vi "bnal PLOT_NS.vi"(7 "AS IDX":i32[](array[numeric]), 8 "error in":errorcluster caption="エラー入力（エラーなし）", 9 "Signal Intensity [pA]":dbl[](array[numeric]), 10 "Time":dbl[](array[numeric]), 11 "Relative Averaged Data":dbl[](array[numeric])) -> (0 "error out":errorcluster caption="エラー出力", 1 "R Con H":dbl[][](array[numeric]), 2 "Plot_C":T2, 3 "Plot Graph":T1)   [LabVIEW 2018]
uses:
  <vilib>/Analysis/NI_AALPro.lvlib
  <vilib>/Analysis/NI_AALBase.lvlib
panel:
  out "x/y":dbl
  out "New MIN":dbl
  out "New MAX 2":dbl
  out "最大値 2":dbl
  out "Histogram":i32[][](array[numeric])
  out "配列 2":dbl[][](array[numeric])
  out "GAT":T3
  out "GAF":T4
  out "Abs MIN 2":dbl
  out "Abs MAX 2":dbl
  out "Axis 2":dbl[](array[numeric])
  out "Abs MIN":dbl
  out "Abs MAX":dbl
  out "Axis":dbl[](array[numeric]) caption="軸" format="%0.2f"
  out "Abs Plot Graph":dbl[][](graph)
  out "Abs Average":dbl[](array[numeric])
  out "Total Con and T":T5
  out "T STD (%)":dbl[](array[numeric])
  out "T Average":dbl[](array[numeric])
  out "New bin":dbl
  out "New MAX":dbl
  out "Count Graph":cluster{i32[], i32[]}(graph) caption="ヒストグラムグラフ"
  out "Normalized Plot Graph":dbl[][](graph)
  out "STD (%)":dbl[](array[numeric])
  out "Average":dbl[](array[numeric])
  out "layer":i32[](array[numeric])
  out "Plot Graph":dbl[][](graph)
  out "配列":dbl[](array[numeric])
  out "Histogram 2":i32[](array[numeric]) caption="ヒストグラム"
  out "最大値":i32
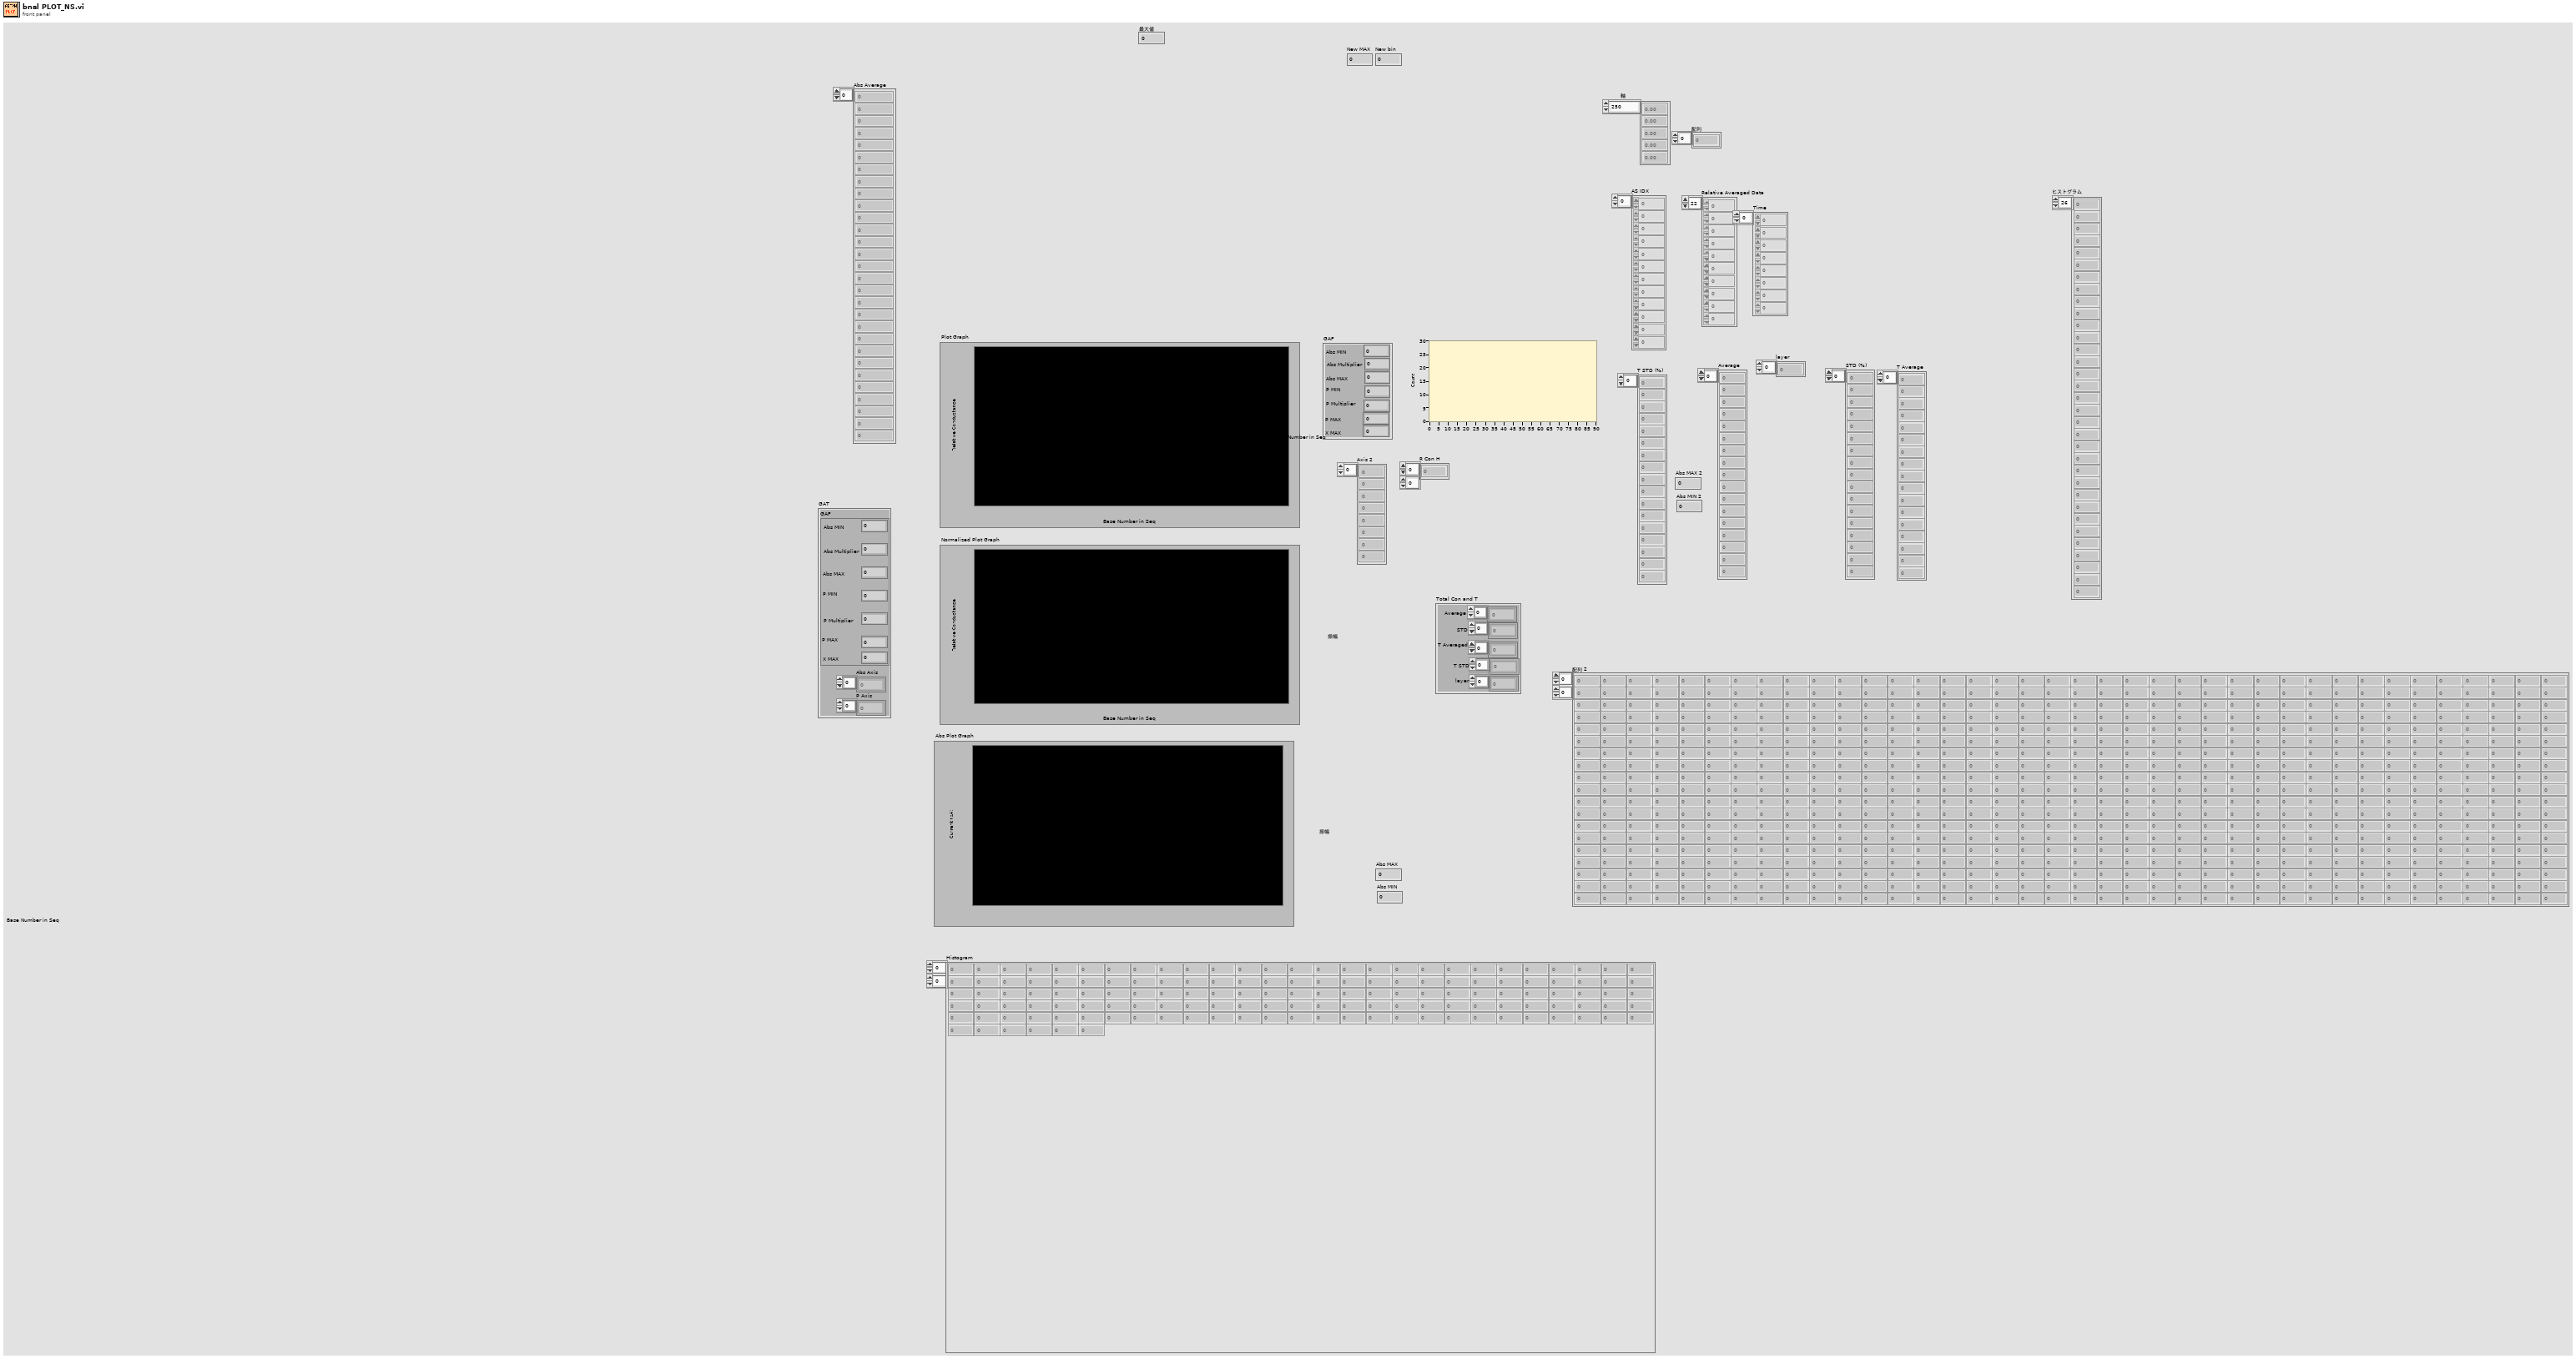
[diagram p1: front panel]
types:
  T1 = cluster{"Plot Graph":dbl[][], "N_Grpah":dbl[][], "Abs_Graph":dbl[][]}
  T2 = cluster{"Count Graph":cluster{i32[], i32[]}, "Total Con and T":cluster{dbl[], dbl[], dbl[], dbl[], i32[]}, "GAT":cluster{"Value":cluster{"Abs MIN":dbl, "Abs Multiplier":dbl, "Abs MAX":dbl, "P MIN":dbl, "P Multiplier":dbl, "P MAX":dbl, "X MAX":dbl}, "Axis":dbl[], "Axis":dbl[]}}
  T3 = cluster{"GAF":cluster{"Abs MIN":dbl, "Abs Multiplier":dbl, "Abs MAX":dbl, "P MIN":dbl, "P Multiplier":dbl, "P MAX":dbl, "X MAX":dbl}, "Abs Axis":dbl[], "P Axis":dbl[]}
  T4 = cluster{"Abs MIN":dbl, "Abs Multiplier":dbl, "Abs MAX":dbl, "P MIN":dbl, "P Multiplier":dbl, "P MAX":dbl, "X MAX":dbl}
  T5 = cluster{"Average":dbl[], "STD":dbl[], "T Averaged":dbl[], "T STD":dbl[], "layer":i32[]}
  T6 = cluster{"Value":cluster{"Abs MIN":dbl, "Abs Multiplier":dbl, "Abs MAX":dbl, "P MIN":dbl, "P Multiplier":dbl, "P MAX":dbl, "X MAX":dbl}, "Axis":dbl[], "Axis":dbl[]}
  T7 = cluster{cluster{i32[], i32[]}, cluster{dbl[], dbl[], dbl[], dbl[], i32[]}, cluster{"Value":cluster{"Abs MIN":dbl, "Abs Multiplier":dbl, "Abs MAX":dbl, "P MIN":dbl, "P Multiplier":dbl, "P MAX":dbl, "X MAX":dbl}, "Axis":dbl[], "Axis":dbl[]}}
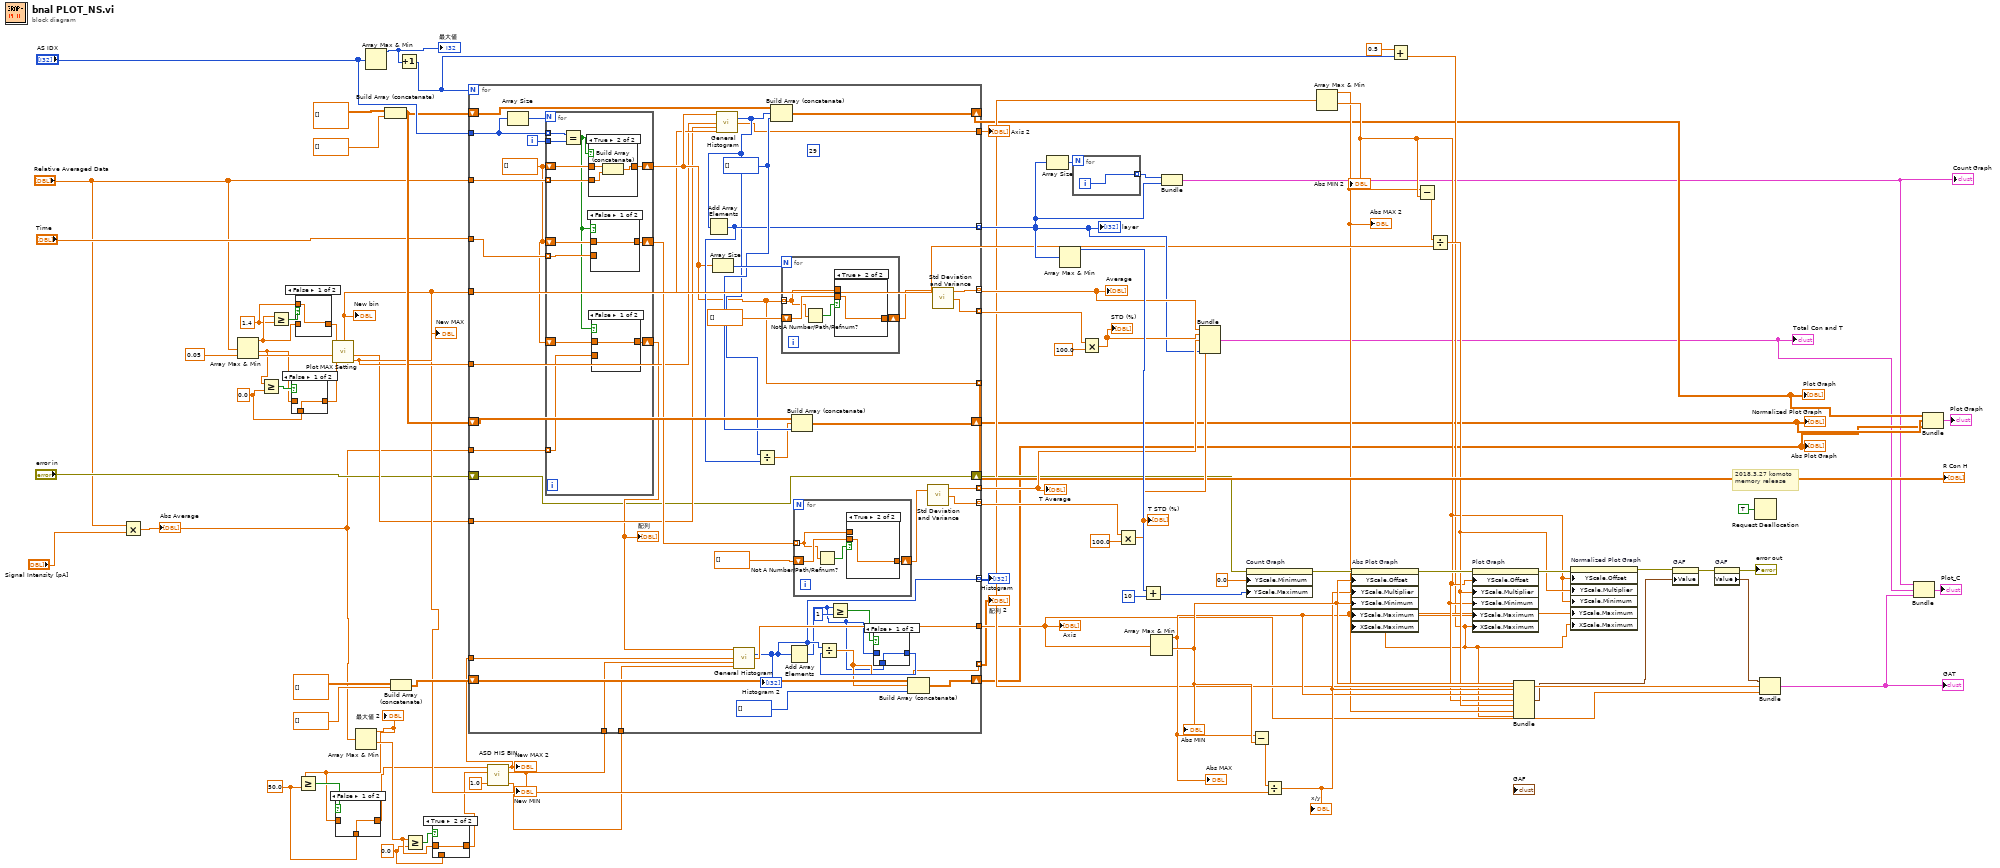
[diagram p0: block diagram]
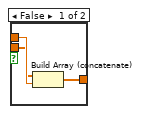
[diagram p7: hidden frame]
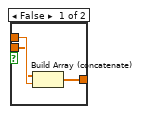
[diagram p8: hidden frame]
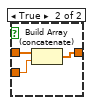
[diagram p9: hidden frame]
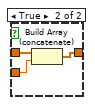
[diagram p10: hidden frame]
diagram:
  w21 = 50.0 ("最大値")
  w25 = 0.0 ("min")
  w31 = 0.0 ("min")
  w32 = 1.4 ("最大値")
  # "2018.3.27 komoto\nmemory release"
  n1 = Multiply(x="Relative Averaged Data", y="Signal Intensity [pA]") -> (x*y=w1:dbl[])
  "Abs Average" <- w1
  n2 = Array Max & Min(array="Relative Averaged Data") -> (max value=w37:dbl, min value=w34:dbl)  [unwired: 2 out]
  n3 = Greater Or Equal?(x=w34, y=w31) -> (x >= y?=w35:bool)
  n4 = Greater Or Equal?(x=w37, y=w32) -> (x >= y?=w38:bool)
  n5 = case shown="False" w35 {
    tunnel: w34 -> [_ w88]
    tunnel: [w87 w88] -> w33
    tunnel: w31 -> [w87 _]
    frame False {
    }
    frame True {
    }
  }
  n6 = case shown="False" w38 {
    tunnel: w37 -> [_ w90]
    tunnel: [w89 w90] -> w36
    tunnel: w32 -> [w89 _]
    frame False {
    }
    frame True {
    }
  }
  n7 = call "Plot MAX Setting.vi"("min"=w33, "bin length"=0.05, "MAX"=w36) -> ("New MAX"=w74:dbl, "New MIN"=w46:dbl, "New bin"=w57:dbl)  [unwired: 6 in]
  "New MAX" <- w74
  "New bin" <- w57
  n8 = Array Max & Min(array=w1) -> (max value=w23:dbl, min value=w26:dbl)  [unwired: 2 out]
  "最大値 2" <- w23
  n9 = Greater Or Equal?(x=w23, y=w21) -> (x >= y?=w24:bool)
  n10 = case shown="False" w24 {
    tunnel: w23 -> [_ w92]
    tunnel: [w91 w92] -> w22
    tunnel: w21 -> [w91 _]
    frame False {
    }
    frame True {
    }
  }
  n11 = Array Max & Min(array="AS IDX") -> (max value=w4:i32)  [unwired: 3 out]
  "最大値" <- w4
  n12 = Build Array (concatenate)(dbl[][] [] ("配列タイプ（2次元Dbl）"), dbl[] [] ("配列")) -> (w81:dbl[][])
  n13 = Build Array (concatenate)(dbl[][] [] ("配列タイプ（2次元Dbl）"), dbl[] [] ("配列")) -> (w62:dbl[][])
  n14 = Increment(x=w4) -> (x+1=w41:i32)
  n15 = Greater Or Equal?(x=w26, y=w25) -> (x >= y?=w28:bool)
  n16 = case shown="True" w28 {
    tunnel: w26 -> [_ w94]
    tunnel: [w93 w94] -> w27
    tunnel: w25 -> [w93 _]
    frame False {
    }
    frame True {
    }
  }
  n17 = call "ASD HIS BIN.vi"("bin length"=1.0, "min"=w27, "MAX"=w22) -> ("New bin"=w48:dbl, "New MIN"=w50:dbl, "New MAX"=w49:dbl)  [unwired: 6 in]
  "New MAX 2" <- w49
  "New MIN" <- w50
  n18 = for {
    N: w41 -> [_]
    tunnel: "Relative Averaged Data" -> [w136]
    tunnel: "AS IDX" -> [w138]
    shift-right: [w135] -> w12
    shift-left: w81 -> [w134]
    tunnel: [w126] -> w66 mode=indexing
    tunnel: [w133] -> w70 mode=indexing
    tunnel: [w132] -> w82 mode=indexing
    shift-right: [w123] -> w11
    shift-left: w81 -> [w128]
    tunnel: w74 -> [w109]
    tunnel: w57 -> [w110]
    tunnel: "Time" -> [w122]
    tunnel: [w121] -> w68 mode=indexing
    tunnel: [w120] -> w71 mode=indexing
    tunnel: [w116] -> w65 mode=indexing
    shift-right: [w114] -> w10
    shift-left: w62 -> [w115]
    tunnel: w1 -> [w113]
    tunnel: w49 -> [w108]
    tunnel: w50 -> [w107]
    tunnel: [w106] -> w52
    tunnel: [w105] -> w53
    tunnel: w48 -> [w104]
    tunnel: w46 -> [w103]
    tunnel: [w98] -> w30 mode=indexing
    tunnel: [w97] -> w29 mode=indexing
    shift-right: [w95] -> w20
    shift-left: "error in" -> [w95]
    i -> [w137]
    w127 = i32[] [] ("配列")
    (unwired) 29 ("# bins")
    w112 = dbl[] []
    n19 = Array Size(array=w138) -> (size(s)=w139:i32)
    n20 = for {
      N: w139 -> [_]
      tunnel: w138 -> [w169] mode=indexing
      tunnel: w137 -> [w168]
      tunnel: w136 -> [w167] mode=indexing
      shift-right: [w165] -> w116
      shift-left: w112 -> [w166]
      tunnel: w122 -> [w164] mode=indexing
      shift-right: [w163] -> w118
      shift-left: w112 -> [w162]
      tunnel: w113 -> [w161] mode=indexing
      shift-right: [w160] -> w99
      shift-left: w112 -> [w159]
      n21 = Equal?(x=w169, y=w168) -> (x = y?=w158:bool)
      n22 = case shown="True" w158 {
        tunnel: w167 -> [_ w181]
        tunnel: [w178 w180] -> w165
        tunnel: w166 -> [w178 w179]
        frame False {
        }
        frame True {
          n23 = Build Array (concatenate)(w179, w181) -> (w180:dbl[])
        }
      }
      n24 = case shown="False" w158 {
        tunnel: w164 -> [_ w177]
        tunnel: [w174 w176] -> w163
        tunnel: w162 -> [w174 w175]
        frame False {
        }
        frame True {
          n25 = Build Array (concatenate)(w175, w177) -> (w176:dbl[])
        }
      }
      n26 = case shown="False" w158 {
        tunnel: w161 -> [_ w173]
        tunnel: [w170 w172] -> w160
        tunnel: w159 -> [w170 w171]
        frame False {
        }
        frame True {
          n27 = Build Array (concatenate)(w171, w173) -> (w172:dbl[])
        }
      }
    }
    "配列" <- w99
    n28 = Array Size(array=w116) -> (size(s)=w131:i32)
    n29 = call <vilib>:"General Histogram.vi"("X"=w116, "max"=w109, "min"=w103, "# bins"=w110) -> ("Histogram"=w125:i32[], "Axis"=w105:dbl[])  [unwired: 7 in, 3 out]
    n30 = Add Array Elements(numeric array=w125) -> (sum=w126:i32)
    n31 = call <vilib>:"General Histogram.vi"("X"=w99, "max"=w108, "min"=w107, "# bins"=w104) -> ("Histogram"=w97:i32[], "Axis"=w106:dbl[])  [unwired: 7 in, 3 out]
    "Histogram 2" <- w97
    n32 = Divide(x=w125, y=w126) -> (x/y=w124:dbl[])
    n33 = Build Array (concatenate)(w134, w125, w127) -> (w135:dbl[][])
    n34 = for {
      N: w131 -> [_]
      tunnel: w116 -> [w151] mode=indexing
      shift-right: [w153] -> w129
      shift-left: dbl[] [] -> [w152]
      n35 = Not A Number/Path/Refnum?(number/path/refnum=w151) -> (NaN/Path/Refnum?=w150:bool)
      n36 = case shown="True" w150 {
        tunnel: w151 -> [w156 _]
        tunnel: [w155 w157] -> w153
        tunnel: w152 -> [w154 w157]
        frame False {
          n37 = Build Array (concatenate)(w154, w156) -> (w155:dbl[])
        }
        frame True {
        }
      }
    }
    n38 = Add Array Elements(numeric array=w97) -> (sum=w96:i32)
    n39 = Build Array (concatenate)(w128, w124, w127) -> (w123:dbl[][])
    n40 = for {
      tunnel: w118 -> [w143] mode=indexing
      shift-right: [w145] -> w117
      shift-left: dbl[] [] ("配列") -> [w144]
      n41 = Not A Number/Path/Refnum?(number/path/refnum=w143) -> (NaN/Path/Refnum?=w142:bool)
      n42 = case shown="True" w142 {
        tunnel: w143 -> [w148 _]
        tunnel: [w147 w149] -> w145
        tunnel: w144 -> [w146 w149]
        frame False {
          n43 = Build Array (concatenate)(w146, w148) -> (w147:dbl[])
        }
        frame True {
        }
      }
    }
    n44 = Greater Or Equal?(x=w96, y=1) -> (x >= y?=w102:bool)
    n45 = case shown="False" w102 {
      tunnel: w96 -> [_ w141]
      tunnel: [w140 w141] -> w100
      tunnel: w96 -> [w140 _]
      frame False {
      }
      frame True {
      }
    }
    n46 = Divide(x=w97, y=w100) -> (x/y=w98:dbl[])
    n47 = Build Array (concatenate)(w115, w98, i32[] [] ("配列")) -> (w114:dbl[][])
    n48 = call <vilib>:"Std Deviation and Variance.vi"("X"=w117) -> ("mean"=w121:dbl, "standard deviation"=w120:dbl)  [unwired: 1 in, 1 out]
    n49 = call <vilib>:"Std Deviation and Variance.vi"("X"=w129) -> ("mean"=w133:dbl, "standard deviation"=w132:dbl)  [unwired: 1 in, 1 out]
  }
  "Plot Graph" <- w12
  "layer" <- w66
  "Average" <- w70
  "Normalized Plot Graph" <- w11
  "T Average" <- w68
  "R Con H" <- w65
  "Abs Plot Graph" <- w10
  "Axis" <- w52
  "Axis 2" <- w53
  "配列 2" <- w30
  "Histogram" <- w29
  n50 = Array Size(array=w66) -> (size(s)=w80:i32)
  n51 = Array Max & Min(array=w66) -> (max value=w78:i32)  [unwired: 3 out]
  n52 = for {
    N: w80 -> [_]
    tunnel: [w182] -> w79 mode=indexing
    i -> [w182]
  }
  n53 = Multiply(x=w82, y=100.0) -> (x*y=w69:dbl[])
  "STD (%)" <- w69
  n54 = Multiply(x=w71, y=100.0) -> (x*y=w67:dbl[])
  "T STD (%)" <- w67
  n55 = Add(x=w78, y=10) -> (x+y=w75:i32)
  n56 = Array Max & Min(array=w52) -> (max value=w54:dbl, min value=w56:dbl)  [unwired: 2 out]
  "Abs MAX" <- w54
  "Abs MIN" <- w56
  n57 = Bundle(w79, w66) -> (w9:cluster{i32[], i32[]})  [unwired: 1 in]
  "Count Graph" <- w9
  n58 = Bundle(w70, w69, w68, w67, w66) -> (w8:cluster{dbl[], dbl[], dbl[], dbl[], i32[]})  [unwired: 1 in]
  "Total Con and T" <- w8
  n59 = property on="Count Graph" class="XYGraph (strict)"(error in=w20, "YScale.Minimum"=0.0 ("Yスケール.範囲:最小値"), "YScale.Maximum"=w75) -> (error out=w61:errorcluster)  [unwired: 1 in, 1 out]
  n60 = Subtract(x=w54, y=w56) -> (x-y=w60:dbl)
  n61 = Divide(x=w60, y=w57) -> (x/y=w55:dbl)
  "x/y" <- w55
  n62 = Array Max & Min(array=w53) -> (max value=w42:dbl, min value=w43:dbl)  [unwired: 2 out]
  "Abs MAX 2" <- w42
  "Abs MIN 2" <- w43
  n63 = Add(x=0.5, y=w41) -> (x+y=w39:dbl)
  n64 = property on="Abs Plot Graph" class="IntGraph (strict)"(error in=w61, "YScale.Offset"=w56, "YScale.Multiplier"=w55, "YScale.Minimum"=w56, "YScale.Maximum"=w54, "XScale.Maximum"=w39) -> (error out=w59:errorcluster)  [unwired: 1 in, 1 out]
  n65 = Subtract(x=w42, y=w43) -> (x-y=w58:dbl)
  n66 = Divide(x=w58, y=w57) -> (x/y=w44:dbl)
  n67 = property on="Plot Graph" class="IntGraph (strict)"(error in=w59, "YScale.Offset"=w43, "YScale.Multiplier"=w44, "YScale.Minimum"=w43, "YScale.Maximum"=w42, "XScale.Maximum"=w39) -> (error out=w45:errorcluster)  [unwired: 1 in, 1 out]
  n68 = Bundle(w56, w55, w54, w43, w44, w42, w39) -> (w18:cluster{dbl, dbl, dbl, dbl, dbl, dbl, dbl})  [unwired: 1 in]
  n69 = property on="Normalized Plot Graph" class="IntGraph (strict)"(error in=w45, "YScale.Offset"=w43, "YScale.Multiplier"=w44, "YScale.Minimum"=w43, "YScale.Maximum"=w42, "XScale.Maximum"=w39) -> (error out=w19:errorcluster)  [unwired: 1 in, 1 out]
  n70 = property on="GAF" class="Clust (strict)"(error in=w19, "Value"=w18) -> (error out=w17:errorcluster)  [unwired: 1 in, 1 out]
  n71 = property on="GAF" class="Clust (strict)"(error in=w17) -> (error out=→"error out":errorcluster, "Value"=w15:T4)  [unwired: 1 in, 1 out]
  n72 = Request Deallocation(TRUE ("フラグ")) -> ()
  n73 = Bundle("Value"=w15, "Axis"=w53, "Axis"=w52) -> (w7:T6)  [unwired: 1 in]
  "GAT" <- w7
  n74 = Bundle(w9, w8, w7) -> (→"Plot_C":T7)  [unwired: 1 in]
  n75 = Bundle(w12, w11, w10) -> (→"Plot Graph":cluster{dbl[][], dbl[][], dbl[][]})  [unwired: 1 in]
